vi "Set_SglVar_BulkMode_Value.vi"(8 "error in (no error)":errorcluster, 9 "varValue":dbl[](array[numeric]) format="%#_13g", 11 "muExpr in":refnum<class "mupExpr.lvclass">) -> (0 "error out":errorcluster, 3 "muExpr out":refnum<class "mupExpr.lvclass">)   [LabVIEW 2015, in "mupExpr.lvclass"]
doc: "Set the bulk mode values of the expression's single variable.\n\nIf the expression contains no variables, the input value is ignored."
uses:
  mupExpr.lvclass
  mupExpr.lvclass/mupExpr.ctl
  mupLib/mupLib.lvlib
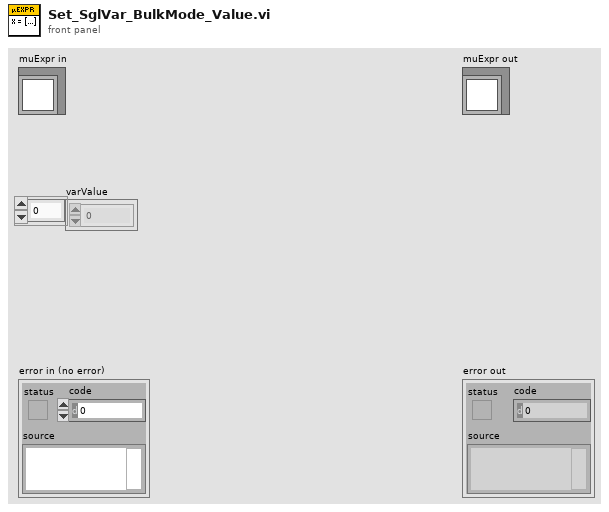
[diagram p1: front panel]
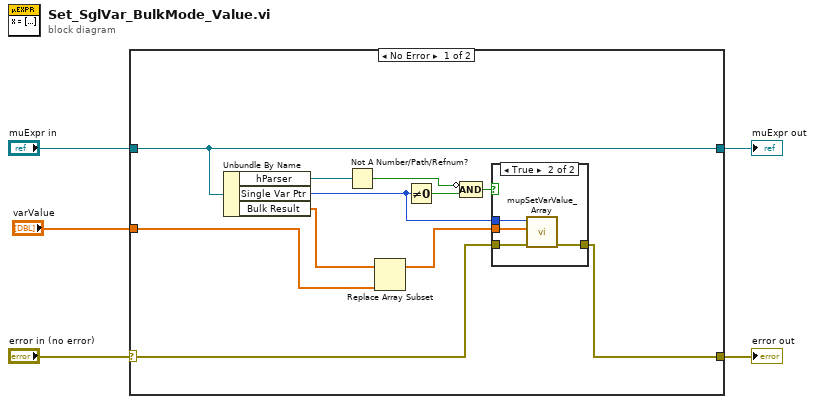
[diagram p0: block diagram]
diagram:
  n1 = case shown="No Error" "error in (no error)" {
    selector: "error in (no error)" -> [w11 w22]
    tunnel: "varValue" -> [w16 _]
    tunnel: "muExpr in" -> [w12 w23]
    tunnel: [w10 w22] -> w3
    tunnel: [w12 w23] -> w2
    frame No Error {
      n2 = Unbundle By Name(w12) -> ("hParser"=w8:refnum<data-value>, "Single Var Ptr"=w15:u64, "Bulk Result"=w14:dbl[])
      n3 = Not A Number/Path/Refnum?(number/path/refnum=w8) -> (NaN/Path/Refnum?=w7:bool)
      n4 = Replace Array Subset(array=w14, new element=w16) -> (w13:dbl[])  [unwired: 1 in]
      n5 = Not Equal To 0?(x=w15) -> (x != 0?=w9:bool)
      n6 = Compound Arithmetic op=AND(invert w7, w9) -> (w6:bool)
      n7 = case shown="True" w6 {
        tunnel: w15 -> [_ w21]
        tunnel: w13 -> [_ w20]
        tunnel: w11 -> [w17 w19]
        tunnel: [w17 w18] -> w10
        frame False {
        }
        frame True {
          n8 = call "mupSetVarValue_Array.vi"("error in (no error)"=w19, "varValue"=w20, "varPtr in"=w21) -> ("error out"=w18:errorcluster)  [unwired: 7 in, 1 out]
        }
      }
    }
    frame Error {
    }
  }
  "error out" <- w3
  "muExpr out" <- w2
